vi "Supplied Panel.vi"() -> ()   [LabVIEW 2026]
doc: "Round-12 graft probe: a supplied PANEL with no diagram at all. Seven terminals, exactly the labels and types of round4's Batch Averager, no nodes - the shape a customer or an exam hands over. The scaffold (Scaffold Scaled.vi) carries the same seven plus one new control, so the graft has to paste the program, replace every duplicated control with the supplied one, and add Scale as a new control."
panel:
  out "Log":string
  out "Average":dbl
  out "Items Processed":i32
  out "Sum":dbl
  out "Final State":T1(ring)
  in  "Items":dbl[](array[numeric])=[1.5, 2.5, 3.5, 4.5]
  in  "Initial State":T1(ring)
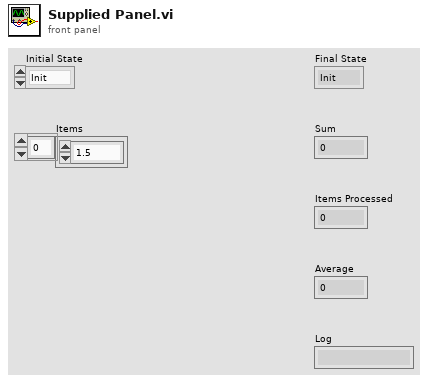
[diagram p1: front panel]
types:
  T1 = enum16{"Init", "Load", "Accumulate", "Report", "Stop"}
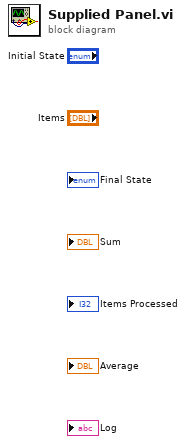
[diagram p0: block diagram]
diagram:
